vi "DVR Get Data.vi"(8 "error in (no error)":errorcluster) -> (0 "error out":errorcluster, 3 "Data":T1)   [LabVIEW 2019, in "Language Selection.lvlib"]
doc: "Converts the Data Value Reference back into Controls translation.\n- - -\nCopyright (c) 2026, Merecs Engineering GmbH"
uses:
  Language Selection.lvlib
  community/Cluster Settings Data.ctl
  Global Language Selection.vi
panel:
  # "Connector Pane"
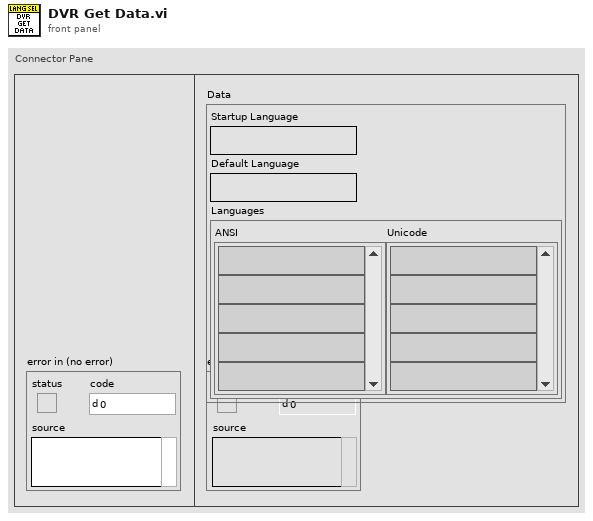
[diagram p1: front panel]
types:
  T1 = typedef "Language Selection.lvlib/Cluster Settings Data.ctl" = cluster{"Startup Language":string, "Default Language":string, "Languages":cluster{"ANSI":string[], "Unicode":string[]}}
  T2 = typedef "Language Selection.lvlib/Cluster DVR.ctl" = cluster{"Data":T1, "VIs":path[], "FP Translation":map{string, T3}, "Text Translation":map{string, T3}, "Front panels":set{refnum<vi>}}
  T3 = typedef "Language Selection.lvlib/Cluster LanguageClusterWithRefnum.ctl" = cluster{"Property":T4[], "Controls":set{refnum<vi>}}
  T4 = typedef "Language Selection.lvlib/Cluster PropertyTranslation.ctl" = cluster{"Type":T5, "Translation ANSI":string[], "Translation Unicode":string[]}
  T5 = typedef "Language Selection.lvlib/Enum Property Type.ctl" = enum16{"NA", "Caption", "String Value", "Boolean Text", "Ring Strings", "1D Array Elements", "2D Array Elements", "(MC)Listbox Header", "(MC)Listbox Items", "Tab Pages Names", "X & Y GraphChart", "Plot Names", "Table Headers", "Table Items", "TipStrip", "Combobox Strings", "Cursor Name", "Tree Col Headers"}
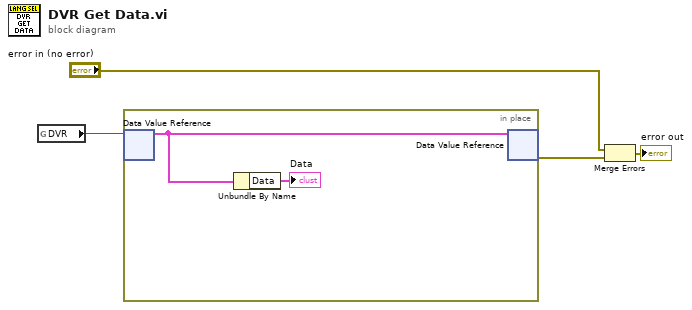
[diagram p0: block diagram]
diagram:
  n1 = global read "Global Language Selection.vi" "DVR"() -> (w1:refnum<data-value>)
  n2 = in-place "In Place Element Structure" {
    n3 = in-place-dvr #1(w1) -> (w6:T2)  [unwired: 1 out]
    n4 = Unbundle By Name(w6) -> ("Data"=→"Data":T1)
    n5 = in-place-dvr #1(w6) -> (w3:errorcluster)  [unwired: 1 out]
  }
  n6 = Merge Errors("error in (no error)", w3) -> (→"error out":errorcluster)
